vi "Analog_Input_Output_Ex.vi"() -> ()   [LabVIEW 2026]
panel:
  in  "Tab Control":enum32{"Read", "Write"}(tab)
  out "Waveform Chart 2":i32(graph)
  out "Waveform Chart":u8(graph)
  in  "Canal Write":u8
  in  "Canal Read":u8
  in  "VISA resource name":refnum<visa-resource-name>
  in  "Stop Button":bool
  out "error out":errorcluster
  # "Ejemplo: Analog Input Output"
  # "Descripción: Lee un pin analógico de entrada y escribe el valor en una salida analógica del microprocesador\n(Solo funcional en microcontroladores con DAC)"
  # "Configuracion"
  # "Indicadores"
  # "Control"
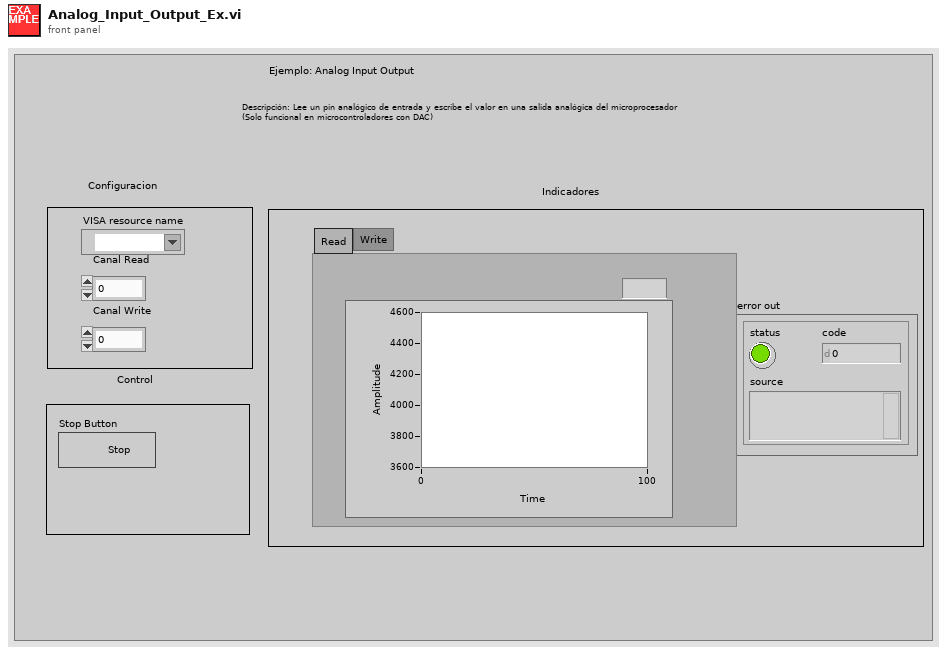
[diagram p1: front panel]
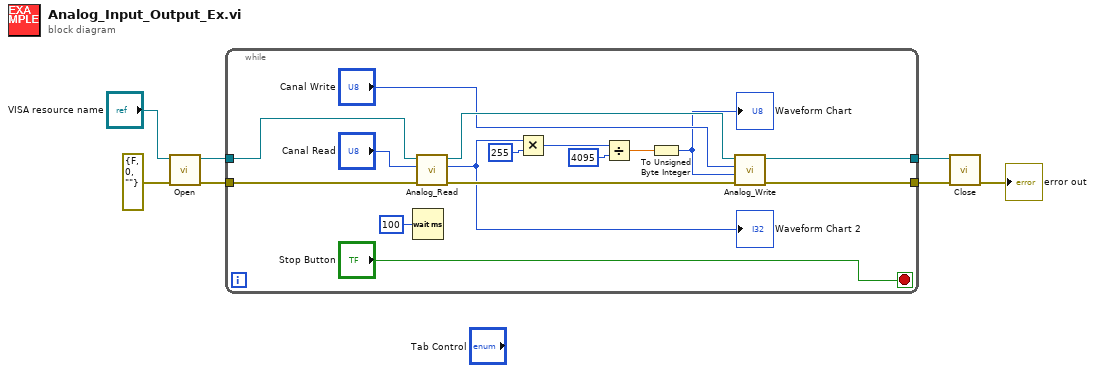
[diagram p0: block diagram]
diagram:
  n1 = call "Open.vi"("error in (no error)"=errorcluster {"status"=FALSE, "code"=0, "source"=""}, "VISA resource name"="VISA resource name") -> ("error out"=w7:errorcluster, "VISA resource name out"=w6:refnum<visa-resource-name>)  [unwired: 8 in]
  n2 = while {
    tunnel: w6 -> [w22]
    tunnel: w7 -> [w21]
    tunnel: [w18] -> w2
    tunnel: [w17] -> w1
    stop <- "Stop Button" stop-if-true
    n3 = Wait (ms)(milliseconds to wait=u32 100) -> ()  [unwired: 1 out]
    n4 = call "Analog_Read.vi"("error in (no error)"=w21, "Canal"="Canal Read", "VISA resource name"=w22) -> ("error out"=w19:errorcluster, "Out"=w10:i32, "VISA resource name out"=w20:refnum<visa-resource-name>)  [unwired: 6 in]
    "Waveform Chart 2" <- w10
    n5 = Multiply(x=w10, y=255) -> (x*y=w13:i32)
    n6 = Divide(x=w13, y=4095) -> (x/y=w11:dbl)
    n7 = To Unsigned Byte Integer(number=w11) -> (unsigned 8bit integer=w9:u8)
    "Waveform Chart" <- w9
    n8 = call "Analog_Write.vi"("error in (no error)"=w19, "Valor"=w9, "Canal"="Canal Write", "VISA resource name"=w20) -> ("error out"=w17:errorcluster, "VISA resource name out"=w18:refnum<visa-resource-name>)  [unwired: 6 in]
  }
  n9 = call "Close.vi"("error in (no error)"=w1, "VISA resource name"=w2) -> ("error out"=→"error out":errorcluster)  [unwired: 9 in]
